vi "Programa Caracterizacion Oleds.vi"() -> ()   [LabVIEW 2020]
uses:
  <vilib>/Instr/_visa.llb/VISA Configure Serial Port (Instr).vi
  <vilib>/Utility/file.llb/Write To Spreadsheet File (string).vi
panel:
  in  "milliseconds to wait":u32
  out "Eficiencia luminosa-V":cluster{dbl[], dbl[]}(graph) caption="L-V"
  out "Eficiencia de corriente-V":cluster{dbl[], dbl[]}(graph) caption="L-V"
  in  "Integration Time (6000)":u32=6000
  in  "Puerto serial Fuente":refnum<visa-resource-name>="COM1"
  out "J-V":cluster{dbl[], dbl[]}(graph)
  out "L-V":cluster{dbl[], dbl[]}(graph)
  in  "Area del OLED [cm2]":dbl
  in  "Distancia OLED-fotodiodo [cm]":dbl
  out "Iluminancia":dbl
  out "Pin":dbl
  out "Analog Vout":dbl
  out "Eficiencia luminosa":dbl
  in  "Color de emisión":u16(ring) items=["Violeta(360-450nm)", "Azul(450-500nm)", "Verde (500-570nm)", "Amarillo (570-590nm)", "Naranja (590-610)", "Rojo (610-670nm)", "Blanco"]
  out "Luminancia":dbl
  in  "Corriente de Proteccion [A]\n(0.1-0.3A recomendado)":dbl=0.1
  in  "Inicio de Barrido (V)":dbl
  in  "Voltaje máximo [V]\n(20V max. recomendado)":dbl=10.0
  in  "Iniciar":bool
  in  "Numero de pasos\n(100-250 recomendado)":dbl=100.0
  in  "Exit":bool
  # "Sistema de caracterización de OLEDs"
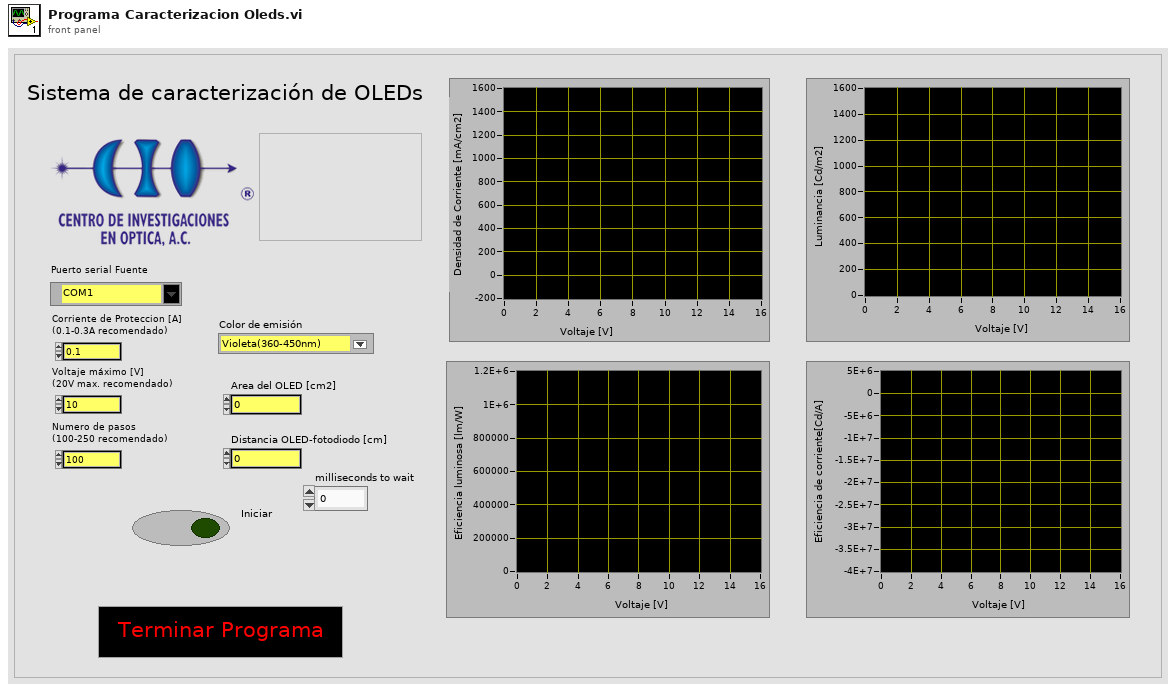
[diagram p1: front panel]
types:
  T1 = enum16{"Parametros", "Procesamiento", "Voltage", "Guardar"}
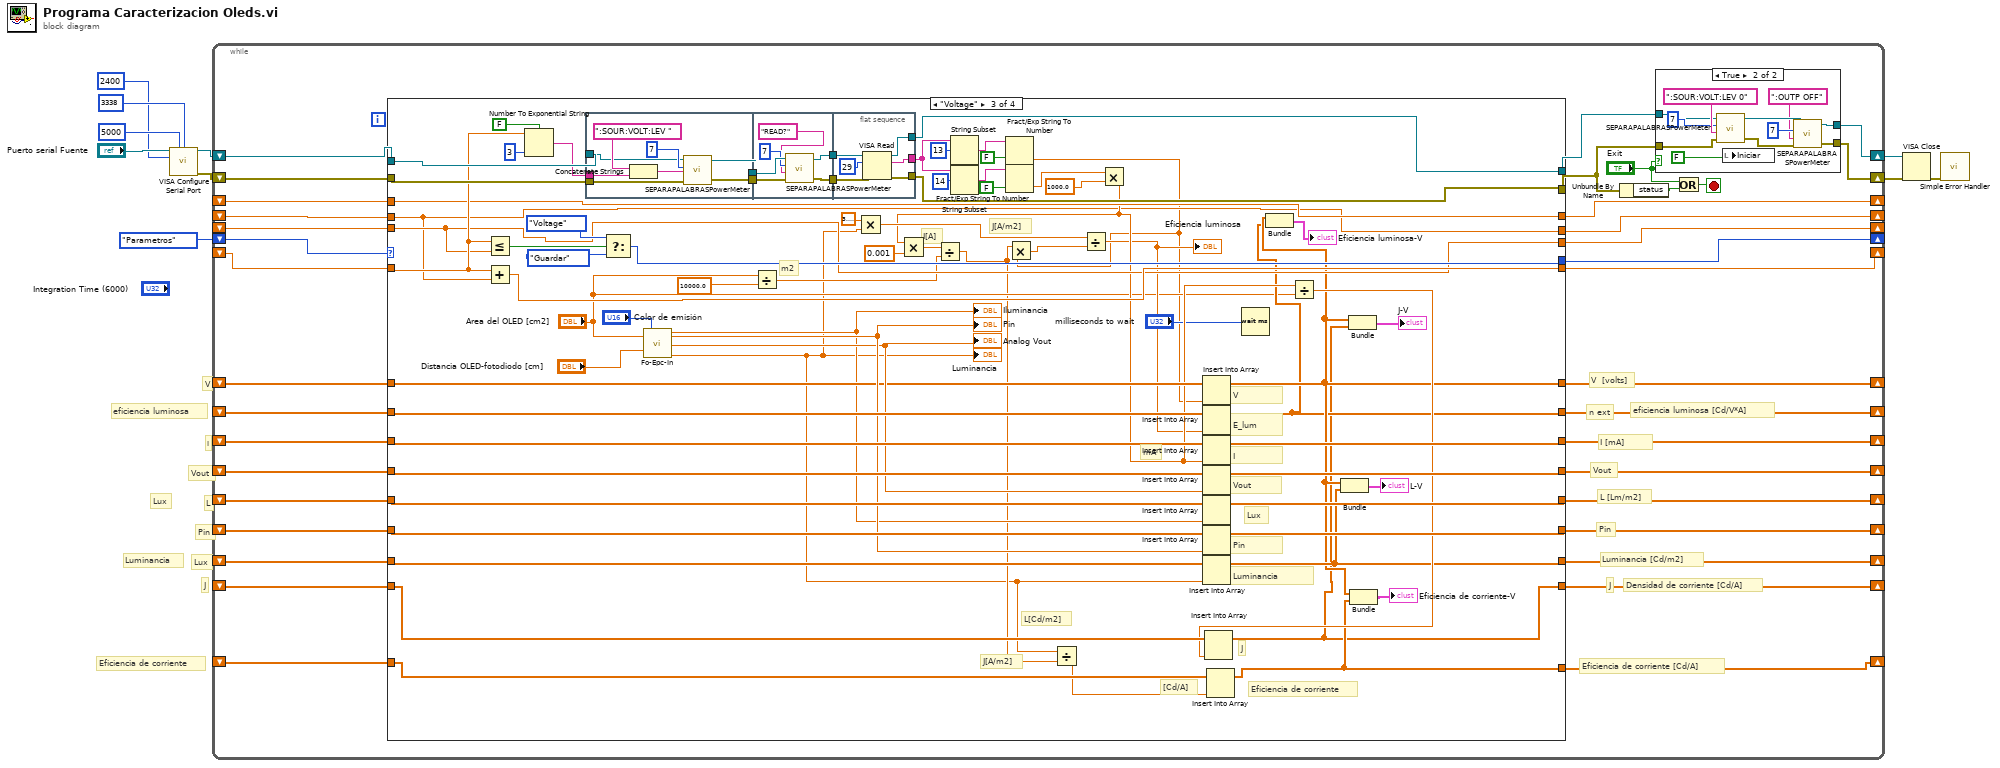
[diagram p0: block diagram]
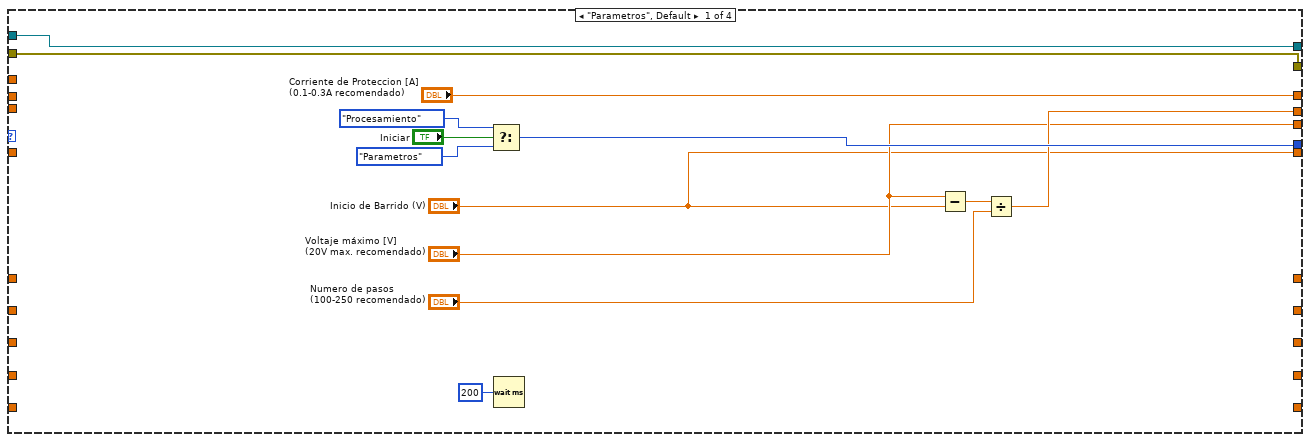
[diagram p3: hidden frame]
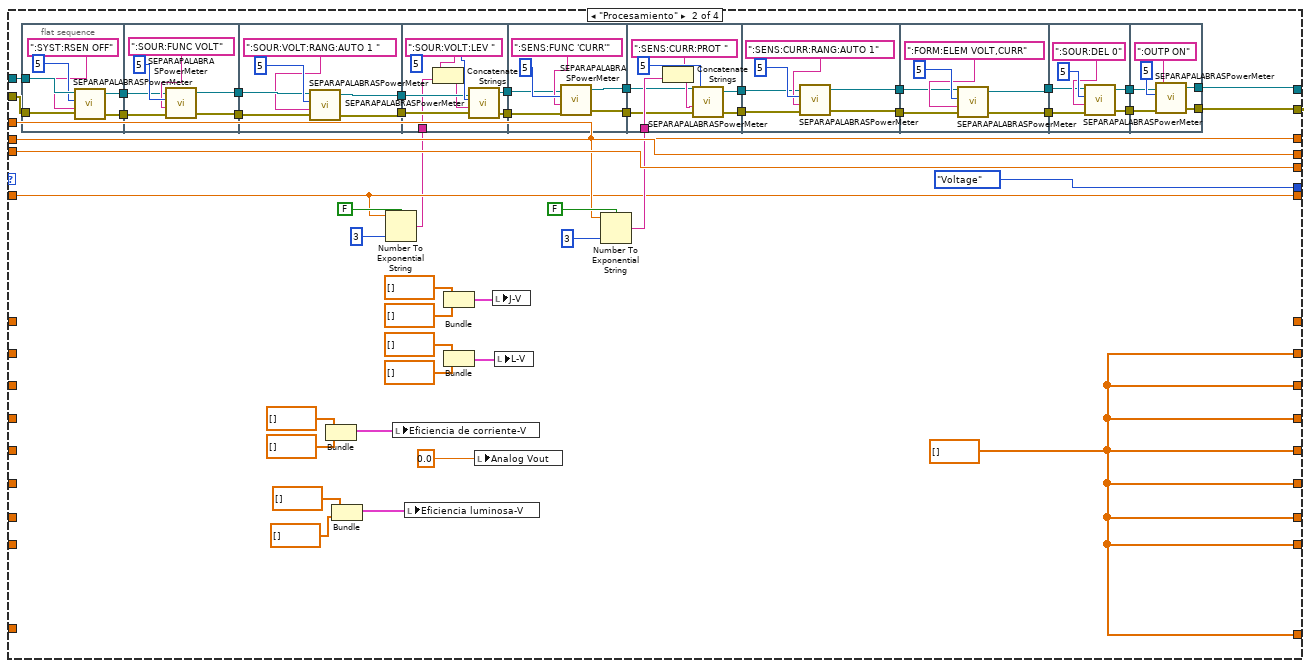
[diagram p4: hidden frame]
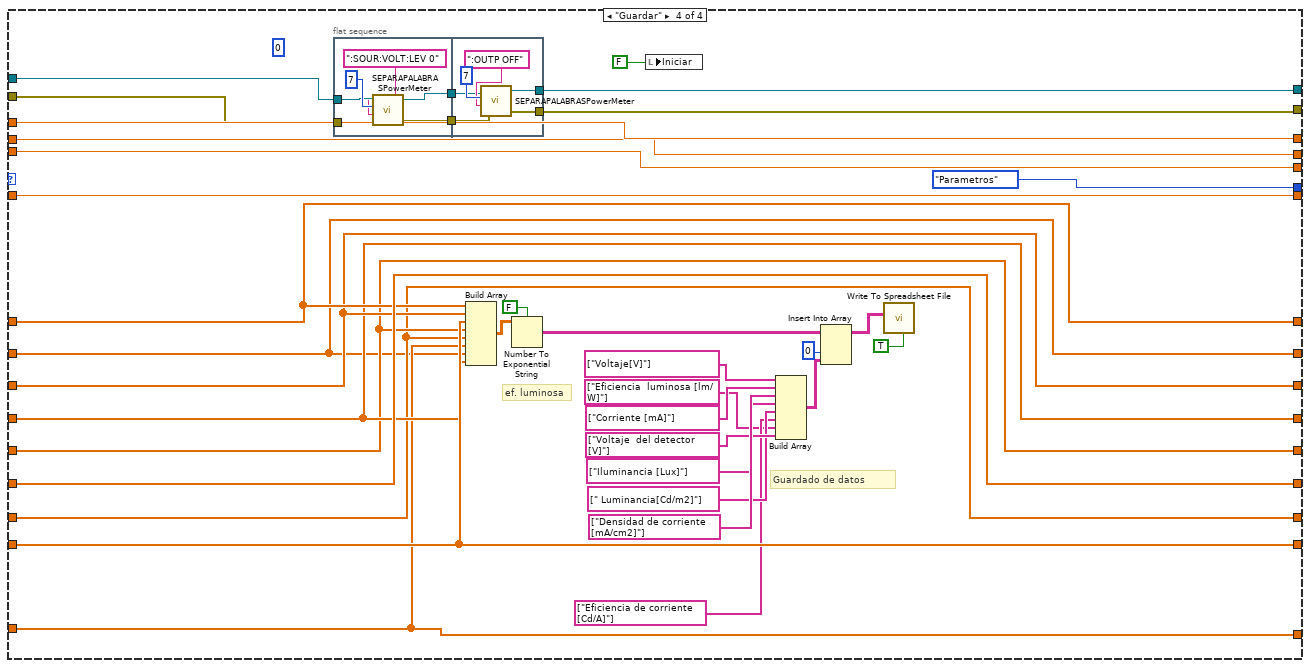
[diagram p5: hidden frame]
diagram:
  # "Eficiencia de corriente"
  # "Luminancia"
  # "Lux"
  # "J"
  # "eficiencia luminosa"
  # "I"
  # "V"
  # "Vout"
  # "L"
  # "Pin"
  # "Lux"
  n1 = call-poly "VISA Configure Serial Port"("VISA resource name"="Puerto serial Fuente", "timeout (10sec)"=u32 5000, "termination char\n(0xA = '\\n' = LF)"=u16 3338 ("termination char\n(0xA = '\\n' = LF)"), "baud rate (9600)"=u32 2400) -> ("VISA resource name out"=w5:refnum<visa-resource-name>, "error out"=w4:errorcluster)  [unwired: 4 in, 6 out]
  n2 = while {
    shift-right: [w44] -> _
    shift-left: T1."Parametros" -> [w47]
    shift-right: [w30] -> w8
    shift-left: w5 -> [w46]
    shift-right: [w29] -> w7
    shift-left: w4 -> [w45]
    shift-right: [w41] -> _
    shift-left: _ -> [w39]
    shift-right: [w40] -> _
    shift-left: _ -> [w38]
    shift-right: [w11] -> _
    shift-left: _ -> [w37]
    shift-right: [w36] -> _
    shift-left: _ -> [w35]
    shift-right: [w32] -> _
    shift-left: _ -> [w25]
    shift-right: [w33] -> _
    shift-left: _ -> [w34]
    shift-right: [w27] -> _
    shift-left: _ -> [w26]
    shift-right: [w22] -> _
    shift-left: _ -> [w21]
    shift-right: [w23] -> _
    shift-left: _ -> [w20]
    shift-right: [w19] -> _
    shift-left: _ -> [w18]
    shift-right: [w17] -> _
    shift-left: _ -> [w16]
    shift-right: [w14] -> _
    shift-left: _ -> [w15]
    shift-right: [w12] -> _
    shift-left: _ -> [w13]
    stop <- w42 stop-if-true
    # "Densidad de corriente [Cd/A]"
    # "eficiencia luminosa [Cd/V*A]"
    # "Eficiencia de corriente [Cd/A]"
    # "J"
    # "Luminancia [Cd/m2]"
    # "Pin"
    # "L [Lm/m2]"
    # "Vout"
    # "I [mA]"
    # "n ext"
    # "V  [volts]"
    n3 = case shown="\"Voltage\"" w47 {
      tunnel: w46 -> [w63 w120 w256 w308]
      tunnel: w45 -> [w69 w119 w231 w307]
      tunnel: [w70 T1."Voltage" w247 T1."Parametros"] -> w44
      tunnel: [w63 w110 w220 w306] -> w31
      tunnel: [w69 w109 w252 w305] -> w24
      tunnel: ["Inicio de Barrido (V)" w90 w251 w312] -> w41
      tunnel: ["Voltaje máximo [V]\n(20V max. recomendado)" w108 w219 w295] -> w40
      tunnel: [w67 w107 w187 w294] -> w11
      tunnel: w39 -> [_ w90 w230 w312]
      tunnel: w38 -> [_ w108 w219 w295]
      tunnel: w37 -> [_ w107 w187 w294]
      tunnel: ["Corriente de Proteccion [A]\n(0.1-0.3A recomendado)" w103 w213 w311] -> w36
      tunnel: w35 -> [_ w103 w213 w311]
      tunnel: w25 -> [_ _ w232 w277]
      tunnel: w34 -> [_ _ w233 w289]
      tunnel: [_ w77 w208 w289] -> w33
      tunnel: [_ w77 w196 w277] -> w32
      tunnel: [_ w77 w228 w285] -> w27
      tunnel: w26 -> [_ _ w224 w285]
      tunnel: [_ w77 w209 w283] -> w23
      tunnel: [_ w77 w229 w293] -> w22
      tunnel: w21 -> [_ _ w226 w293]
      tunnel: w20 -> [_ _ w225 w283]
      tunnel: [_ w77 w202 w281] -> w19
      tunnel: w18 -> [_ _ w227 w281]
      tunnel: [_ _ w198 w291] -> w17
      tunnel: w16 -> [_ _ w217 w291]
      tunnel: w15 -> [_ _ w207 w287]
      tunnel: [_ w77 w194 w287] -> w14
      tunnel: w13 -> [_ _ w204 w279]
      tunnel: [_ w77 w199 w279] -> w12
      frame "Parametros", Default {
        n4 = Select(t=enum16{"Parametros", "Procesamiento"}."Procesamiento", s="Iniciar", f=enum16{"Parametros", "Procesamiento"}."Parametros") -> (s? t:f=w70:enum16{"Parametros", "Procesamiento"})
        n5 = Wait (ms)(milliseconds to wait=u32 200) -> ()  [unwired: 1 out]
        n6 = Subtract(x="Voltaje máximo [V]\n(20V max. recomendado)", y="Inicio de Barrido (V)") -> (x-y=w68:dbl)
        n7 = Divide(x=w68, y="Numero de pasos\n(100-250 recomendado)") -> (x/y=w67:dbl)
      }
      frame "Procesamiento" {
        w77 = dbl[] []
        n8 = flat-sequence {
          tunnel: w120 -> [w126]
          tunnel: w119 -> [w125]
          tunnel: [w122] -> w118
          tunnel: [w121] -> w117
          tunnel: w118 -> [w130]
          tunnel: w117 -> [w129]
          tunnel: [w128] -> w116
          tunnel: [w127] -> w115
          tunnel: w116 -> [w137]
          tunnel: w115 -> [w136]
          tunnel: [w135] -> w114
          tunnel: [w134] -> w113
          tunnel: w114 -> [w145]
          tunnel: w113 -> [w144]
          tunnel: [w143] -> w101
          tunnel: [w142] -> w100
          tunnel: w89 -> [w140]
          tunnel: w101 -> [w149]
          tunnel: w100 -> [w150]
          tunnel: [w148] -> w99
          tunnel: [w147] -> w98
          tunnel: w105 -> [w157]
          tunnel: w99 -> [w156]
          tunnel: w98 -> [w155]
          tunnel: [w154] -> w97
          tunnel: [w153] -> w96
          tunnel: [w165] -> w112
          tunnel: [w164] -> w111
          tunnel: w97 -> [w162]
          tunnel: w96 -> [w161]
          tunnel: w112 -> [w170]
          tunnel: w111 -> [w169]
          tunnel: [w168] -> w88
          tunnel: [w167] -> w87
          tunnel: w88 -> [w176]
          tunnel: w87 -> [w175]
          tunnel: [w174] -> w86
          tunnel: [w173] -> w85
          tunnel: w86 -> [w180]
          tunnel: w85 -> [w179]
          tunnel: [w182] -> w110
          tunnel: [w181] -> w109
          frame #0 {
            n9 = call "SEPARAPALABRASPowerMeter.VI"("error in"=w125, "Comando"=":SYST:RSEN OFF", "Tiempo de espera"=u32 5, "VISA resource name in"=w126) -> ("error out"=w122:errorcluster, "VISA resource name out"=w121:refnum<visa-resource-name>)  [unwired: 1 out]
          }
          frame #1 {
            n10 = call "SEPARAPALABRASPowerMeter.VI"("error in"=w130, "Comando"=":SOUR:FUNC VOLT", "Tiempo de espera"=u32 5, "VISA resource name in"=w129) -> ("error out"=w128:errorcluster, "VISA resource name out"=w127:refnum<visa-resource-name>)  [unwired: 1 out]
          }
          frame #2 {
            n11 = call "SEPARAPALABRASPowerMeter.VI"("error in"=w137, "Comando"=":SOUR:VOLT:RANG:AUTO 1 ", "Tiempo de espera"=u32 5, "VISA resource name in"=w136) -> ("error out"=w134:errorcluster, "VISA resource name out"=w135:refnum<visa-resource-name>)  [unwired: 1 out]
          }
          frame #3 {
            n12 = Concatenate Strings(":SOUR:VOLT:LEV " ("Comando"), w140) -> (w139:string)
            n13 = call "SEPARAPALABRASPowerMeter.VI"("error in"=w144, "Comando"=w139, "Tiempo de espera"=u32 5, "VISA resource name in"=w145) -> ("error out"=w143:errorcluster, "VISA resource name out"=w142:refnum<visa-resource-name>)  [unwired: 1 out]
          }
          frame #4 {
            n14 = call "SEPARAPALABRASPowerMeter.VI"("error in"=w149, "Comando"=":SENS:FUNC 'CURR'", "Tiempo de espera"=u32 5, "VISA resource name in"=w150) -> ("error out"=w147:errorcluster, "VISA resource name out"=w148:refnum<visa-resource-name>)  [unwired: 1 out]
          }
          frame #5 {
            n15 = Concatenate Strings(":SENS:CURR:PROT " ("Comando"), w157) -> (w158:string)
            n16 = call "SEPARAPALABRASPowerMeter.VI"("error in"=w155, "Comando"=w158, "Tiempo de espera"=u32 5, "VISA resource name in"=w156) -> ("error out"=w153:errorcluster, "VISA resource name out"=w154:refnum<visa-resource-name>)  [unwired: 1 out]
          }
          frame #6 {
            n17 = call "SEPARAPALABRASPowerMeter.VI"("error in"=w161, "Comando"=":SENS:CURR:RANG:AUTO 1", "Tiempo de espera"=u32 5, "VISA resource name in"=w162) -> ("error out"=w164:errorcluster, "VISA resource name out"=w165:refnum<visa-resource-name>)  [unwired: 1 out]
          }
          frame #7 {
            n18 = call "SEPARAPALABRASPowerMeter.VI"("error in"=w169, "Comando"=":FORM:ELEM VOLT,CURR", "Tiempo de espera"=u32 5, "VISA resource name in"=w170) -> ("error out"=w167:errorcluster, "VISA resource name out"=w168:refnum<visa-resource-name>)  [unwired: 1 out]
          }
          frame #8 {
            n19 = call "SEPARAPALABRASPowerMeter.VI"("error in"=w175, "Comando"=":SOUR:DEL 0", "Tiempo de espera"=u32 5, "VISA resource name in"=w176) -> ("error out"=w173:errorcluster, "VISA resource name out"=w174:refnum<visa-resource-name>)  [unwired: 1 out]
          }
          frame #9 {
            n20 = call "SEPARAPALABRASPowerMeter.VI"("error in"=w179, "Comando"=":OUTP ON", "Tiempo de espera"=u32 5, "VISA resource name in"=w180) -> ("error out"=w181:errorcluster, "VISA resource name out"=w182:refnum<visa-resource-name>)  [unwired: 1 out]
          }
        }
        n21 = Bundle(dbl[] [], dbl[] []) -> (w78:cluster{dbl[], dbl[]})  [unwired: 1 out]
        n22 = Bundle(dbl[] [], dbl[] []) -> (w75:cluster{dbl[], dbl[]})  [unwired: 1 out]
        n23 = Number To Exponential String(number=w90, precision (6)=i16 3, 1:FALSE ("use system decimal point (T)")) -> (E-format string=w89:string)  [unwired: 1 out]
        n24 = local write "Eficiencia de corriente-V"(w78) -> ()
        n25 = local write "Eficiencia luminosa-V"(w75) -> ()
        n26 = Bundle(dbl[] [], dbl[] []) -> (w93:cluster{dbl[], dbl[]})  [unwired: 1 out]
        n27 = Bundle(dbl[] [], dbl[] []) -> (w82:cluster{dbl[], dbl[]})  [unwired: 1 out]
        n28 = local write "Analog Vout"(0.0 ("Analog Vout")) -> ()
        n29 = local write "J-V"(w93) -> ()
        n30 = local write "L-V"(w82) -> ()
        n31 = Number To Exponential String(number=w103, precision (6)=i16 3, 1:FALSE ("use system decimal point (T)")) -> (E-format string=w105:string)  [unwired: 1 out]
      }
      frame "Voltage" {
        # "[Cd/A]"
        # "L[Cd/m2]"
        # "J[A/m2]"
        # "m2"
        # "mA"
        # "Eficiencia de corriente"
        # "J"
        # "J[A/m2]"
        # "I[A]"
        # "E_lum"
        # "V"
        # "I"
        # "Vout"
        # "Luminancia"
        # "Pin"
        # "Lux"
        n32 = Less Or Equal?(x=w230, y=w219) -> (x <= y?=w250:bool)
        n33 = Add(x=w230, y=w187) -> (x+y=w251:dbl)
        n34 = Number To Exponential String(number=w230, precision (6)=i16 3, 1:FALSE ("use system decimal point (T)")) -> (E-format string=w253:string)  [unwired: 1 out]
        n35 = flat-sequence {
          tunnel: w256 -> [w261]
          tunnel: w231 -> [w260]
          tunnel: w253 -> [w257]
          tunnel: [w259] -> w239
          tunnel: [w258] -> w238
          tunnel: w239 -> [w270]
          tunnel: w238 -> [w269]
          tunnel: [w266] -> w237
          tunnel: [w265] -> w236
          tunnel: w237 -> [w273]
          tunnel: w236 -> [w272]
          tunnel: [w276] -> w220
          tunnel: [w275] -> w252
          tunnel: [w274] -> w245
          frame #0 {
            n36 = Concatenate Strings(":SOUR:VOLT:LEV " ("Comando"), w257) -> (w262:string)
            n37 = call "SEPARAPALABRASPowerMeter.VI"("error in"=w260, "Comando"=w262, "Tiempo de espera"=u32 7, "VISA resource name in"=w261) -> ("error out"=w258:errorcluster, "VISA resource name out"=w259:refnum<visa-resource-name>)  [unwired: 1 out]
          }
          frame #1 {
            n38 = call "SEPARAPALABRASPowerMeter.VI"("error in"=w269, "Comando"="READ?", "Tiempo de espera"=u32 7, "VISA resource name in"=w270) -> ("error out"=w265:errorcluster, "VISA resource name out"=w266:refnum<visa-resource-name>)  [unwired: 1 out]
          }
          frame #2 {
            n39 = VISA Read(VISA resource name=w273, byte count=u32 29, error in (no error)=w272) -> (VISA resource name out=w276:refnum<visa-resource-name>, read buffer=w274:string, error out=w275:errorcluster)  [unwired: 1 out]
          }
        }
        n40 = Select(t=T1."Voltage", s=w250, f=T1."Guardar") -> (s? t:f=w247:T1)
        n41 = call "Fo-Epc-In.vi"("As (Area del OLED) m2"="Area del OLED [cm2]", "S (Distancia OLED-fotodiodo) m"="Distancia OLED-fotodiodo [cm]", "Color"="Color de emisión") -> ("Iluminancia (lm/m2)"=w216:dbl, "Pin"=w221:dbl, "Analog Vout"=w218:dbl, "Luminancia (Cd/m2)"=w185:dbl)  [unwired: 5 in, 8 out]
        "Iluminancia" <- w216
        "Pin" <- w221
        "Analog Vout" <- w218
        "Luminancia" <- w185
        n42 = Divide(x="Area del OLED [cm2]", y=10000.0) -> (x/y=w190:dbl)
        n43 = Multiply(x=3.141592653589793, y=w185) -> (x*y=w211:dbl)
        n44 = String Subset(string=w245, length (rest)=13 ("length (rest)")) -> (substring=w243:string)  [unwired: 1 out]
        n45 = String Subset(string=w245, offset (0)=14) -> (substring=w241:string)  [unwired: 1 out]
        n46 = Fract/Exp String To Number(use system decimal point (T)=FALSE, string=w243) -> (number=w186:dbl)  [unwired: 3 out]
        n47 = Fract/Exp String To Number(use system decimal point (T)=FALSE, string=w241) -> (number=w235:dbl)  [unwired: 3 out]
        n48 = Multiply(x=w235, y=1000.0) -> (x*y=w205:dbl)
        n49 = Multiply(x=w205, y=0.001) -> (x*y=w212:dbl)
        n50 = Divide(x=w212, y=w190) -> (x/y=w189:dbl)
        n51 = Multiply(x=w189, y=w186) -> (x*y=w206:dbl)
        n52 = Divide(x=w185, y=w189) -> (x/y=w201:dbl)
        n53 = Divide(x=w211, y=w206) -> (x/y=w197:dbl)
        "Eficiencia luminosa" <- w197
        n54 = Insert Into Array(array=w217, new element=w186) -> (w198:dbl[])  [unwired: 1 in]
        n55 = Insert Into Array(array=w232, new element=w197) -> (w196:dbl[])  [unwired: 1 in]
        n56 = Insert Into Array(array=w233, new element=w205) -> (w208:dbl[])  [unwired: 1 in]
        n57 = Insert Into Array(array=w224, new element=w218) -> (w228:dbl[])  [unwired: 1 in]
        n58 = Insert Into Array(array=w225, new element=w216) -> (w209:dbl[])  [unwired: 1 in]
        n59 = Insert Into Array(array=w226, new element=w221) -> (w229:dbl[])  [unwired: 1 in]
        n60 = Insert Into Array(array=w227, new element=w185) -> (w202:dbl[])  [unwired: 1 in]
        n61 = Insert Into Array(array=w204, new element=w201) -> (w199:dbl[])  [unwired: 1 in]
        n62 = Wait (ms)(milliseconds to wait="milliseconds to wait") -> ()  [unwired: 1 out]
        n63 = Bundle(w198, w196) -> (→"Eficiencia luminosa-V":cluster{dbl[], dbl[]})  [unwired: 1 out]
        n64 = Divide(x=w205, y="Area del OLED [cm2]") -> (x/y=w203:dbl)
        n65 = Insert Into Array(array=w207, new element=w203) -> (w194:dbl[])  [unwired: 1 in]
        n66 = Bundle(w198, w202) -> (→"L-V":cluster{dbl[], dbl[]})  [unwired: 1 out]
        n67 = Bundle(w198, w194) -> (→"J-V":cluster{dbl[], dbl[]})  [unwired: 1 out]
        n68 = Bundle(w198, w199) -> (→"Eficiencia de corriente-V":cluster{dbl[], dbl[]})  [unwired: 1 out]
      }
      frame "Guardar" {
        (unwired) 0 ("index (row)")
        # "ef. luminosa"
        # "Guardado de datos"
        n69 = flat-sequence {
          tunnel: w307 -> [w316]
          tunnel: w308 -> [w317]
          tunnel: [w315] -> w301
          tunnel: [w314] -> w300
          tunnel: [w320] -> w306
          tunnel: [w319] -> w305
          tunnel: w301 -> [w322]
          tunnel: w300 -> [w321]
          frame #0 {
            n70 = call "SEPARAPALABRASPowerMeter.VI"("error in"=w316, "Comando"=":SOUR:VOLT:LEV 0", "Tiempo de espera"=u32 7, "VISA resource name in"=w317) -> ("error out"=w314:errorcluster, "VISA resource name out"=w315:refnum<visa-resource-name>)  [unwired: 1 out]
          }
          frame #1 {
            n71 = call "SEPARAPALABRASPowerMeter.VI"("error in"=w321, "Comando"=":OUTP OFF", "Tiempo de espera"=u32 7, "VISA resource name in"=w322) -> ("error out"=w319:errorcluster, "VISA resource name out"=w320:refnum<visa-resource-name>)  [unwired: 1 out]
          }
        }
        n72 = Build Array(w291, w289, w287, w283, w281, w279, w277, w285) -> (w304:dbl[][])
        n73 = Number To Exponential String(number=w304, 1:FALSE ("use system decimal point (T)")) -> (E-format string=w299:string[][])  [unwired: 2 out]
        n74 = local write "Iniciar"(FALSE) -> ()
        n75 = Build Array(string[] ["Voltaje[V]"], string[] ["Corriente [mA]"], string[] ["Densidad de corriente [mA/cm2]"], string[] ["Iluminancia [Lux]"], string[] [" Luminancia[Cd/m2]"], string[] ["Eficiencia de corriente [Cd/A]"], string[] ["Eficiencia  luminosa [lm/W]"], string[] ["Voltaje  del detector [V]"]) -> (w298:string[][])
        n76 = Insert Into Array(array=w299, index (col)=0 ("index (row)"), new element=w298) -> (w297:string[][])  [unwired: 1 in]
        n77 = call-poly <vilib>:"Write To Spreadsheet File.vi"("transpose? (no:F)"=TRUE, "2D data"=w297) -> ()  [unwired: 4 in, 3 out]
      }
    }
    n78 = Unbundle By Name(w24) -> ("status"=w43:bool)
    n79 = case shown="True" "Exit" {
      tunnel: w31 -> [w49 w55]
      tunnel: [w49 w54] -> w30
      tunnel: w24 -> [w48 w53]
      tunnel: [w48 w52] -> w29
      frame False {
      }
      frame True {
        n80 = call "SEPARAPALABRASPowerMeter.VI"("error in"=w53, "Comando"=":SOUR:VOLT:LEV 0", "Tiempo de espera"=u32 7, "VISA resource name in"=w55) -> ("error out"=w56:errorcluster, "VISA resource name out"=w57:refnum<visa-resource-name>)  [unwired: 1 out]
        n81 = local write "Iniciar"(FALSE ("Tomar curva IV")) -> ()
        n82 = call "SEPARAPALABRASPowerMeter.VI"("error in"=w56, "Comando"=":OUTP OFF", "Tiempo de espera"=u32 7, "VISA resource name in"=w57) -> ("error out"=w52:errorcluster, "VISA resource name out"=w54:refnum<visa-resource-name>)  [unwired: 1 out]
      }
    }
    n83 = Or(x="Exit", y=w43) -> (x .or. y?=w42:bool)
  }
  n84 = VISA Close(VISA resource name=w8, error in (no error)=w7) -> (error out=w6:errorcluster)
  n85 = call <vilib>:"Simple Error Handler.vi"("error in (no error)"=w6) -> ()  [unwired: 1 in, 8 out]
